vi "Set Plot Axis.vi"(8 "error in (no error)":errorcluster, 9 "Waveform Array":waveform(dbl)[](array[waveform]), 10 "Large Scale threshold":dbl=10.0 format="%#_13g", 11 "Waveform Chart ref":refnum<vi>) -> (0 "error out":errorcluster, 1 "Waveform Array out":waveform(dbl)[](array[waveform]))   [LabVIEW 2021]
doc: "Move each plot to the Y Axis that matches its magnitude according to threshold.\n\n- Small signals on axis 0\n- Large signals on axis 1"
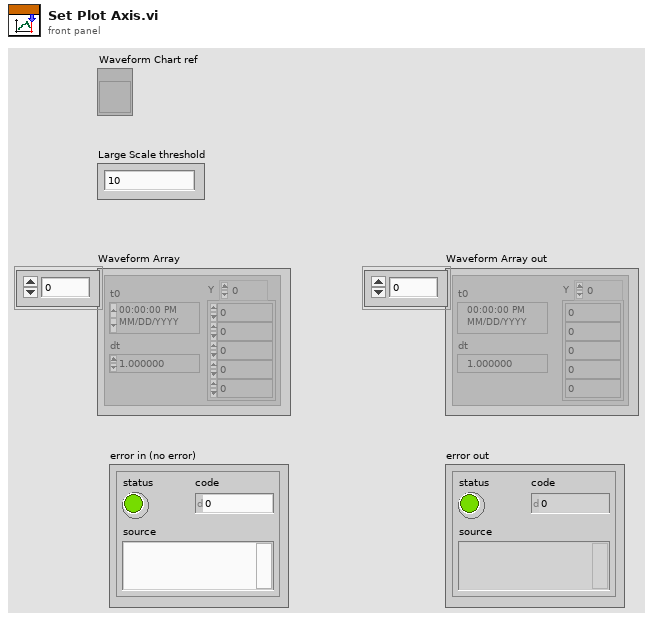
[diagram p1: front panel]
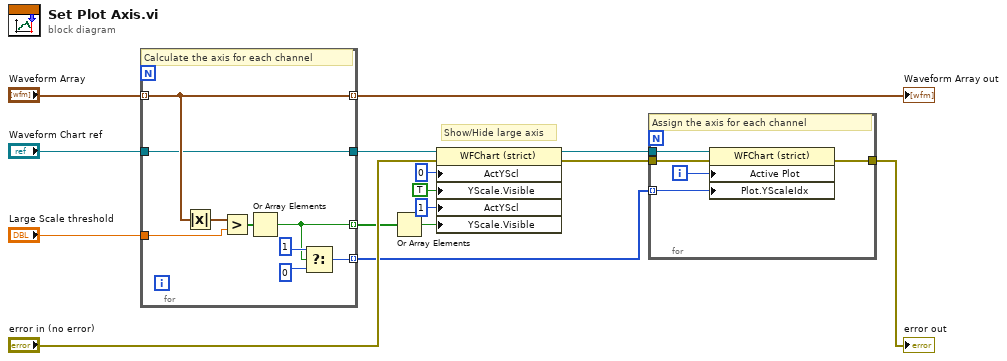
[diagram p0: block diagram]
diagram:
  # "Show/Hide large axis"
  n1 = for {
    tunnel: [w24] -> w15 mode=indexing
    tunnel: "Waveform Array" -> [w24] mode=indexing
    tunnel: "Waveform Chart ref" -> [w16]
    tunnel: [w19] -> w1 mode=indexing
    tunnel: [w16] -> w12
    tunnel: "Large Scale threshold" -> [w18]
    tunnel: [w17] -> w2 mode=indexing
    # "Calculate the axis for each channel"
    n2 = Absolute Value(x=w24) -> (abs(x)=w20:waveform(dbl))
    n3 = Greater?(x=w20, y=w18) -> (0:w23:bool[])
    n4 = Or Array Elements(Boolean array=w23) -> (logical OR=w19:bool)
    n5 = Select(t=u32 1 ("Plot.Y Scale Index"), s=w19, f=u32 0 ("Plot.Y Scale Index")) -> (s? t:f=w17:u32)
  }
  "Waveform Array out" <- w15
  n6 = Or Array Elements(Boolean array=w1) -> (logical OR=w11:bool)
  n7 = property class="WFChart (strict)"(reference=w12, error in="error in (no error)", "ActYScl"=0 ("Active Y Scale"), "YScale.Visible"=TRUE ("Y Scale.Visible"), "ActYScl"=1 ("Active Y Scale"), "YScale.Visible"=w11) -> (reference out=w5:refnum<vi>, error out=w6:errorcluster)
  n8 = for {
    tunnel: w6 -> [w29]
    tunnel: w5 -> [w28]
    tunnel: [w27] -> w4
    tunnel: w2 -> [w25] mode=indexing
    i -> [w26]
    # "Assign the axis for each channel"
    n9 = property class="WFChart (strict)"(reference=w28, error in=w29, "Active Plot"=w26, "Plot.YScaleIdx"=w25) -> (error out=w27:errorcluster)  [unwired: 1 out]
  }
  "error out" <- w4
